vi "Process HTTP Request.vi"(8 "error in":errorcluster, 10 "id in":i32, 11 "Processing in":refnum<class "Processing.lvclass">) -> (0 "error out":errorcluster, 3 "Processing out":refnum<class "Processing.lvclass">)   [LabVIEW 2020, in "MCP Server.lvlib"]
doc: "Answers one HTTP request on the MCP endpoint following the MCP Streamable HTTP transport rules, and stores the response in the Processing object.\n\n1. ACCESS: reads the client host (Get Request, Get Client URI, Get Host: the name from a reverse DNS lookup of the client address), the local address of the connection the request arrived on (Connection Local IP.vi, no DNS) and the Authorization header, and passes them to Check Client Access.vi with the access settings Start.vi stored for this server. \"This computer only\" is decided by that local address; an error reading it only leaves it empty, which Check Client Access.vi refuses in that mode, and never turns into a 500. A client that is not allowed gets 403, a missing or wrong bearer token 401 with WWW-Authenticate: Bearer. These checks win over every later one.\n2. Reads the HTTP method and the Origin and MCP-Protocol-Version request headers and passes them to Validate HTTP Request.vi. Also reads the Mcp-Method and Mcp-Name headers (MCP 2026-07-28).\n3. Rejected request (403, 401, 405 or 400): the MCP server is NOT called. The response carries the status code and the JSON-RPC error payload with Content-Type application/json. A 405 additionally carries the header Allow: POST.\n4. Accepted request: Prepare Request Dispatch.vi answers a legacy notifications/cancelled itself and decides whether a tools/call is streamed (Start Streamed Request.vi). Otherwise the request body, one message or a batch of messages, is passed with the three MCP headers to Handle MCP Request.vi, which decides the era (legacy or modern) per request, makes the modern header checks and answers; its errors are cleared. Its status code is used: 202 with an empty body for a notification, 200 with Content-Type application/json, or 400/404 for a refused modern request.\n\nerror out reports only errors of the first two header reads. It is informational: a response is always set."
uses:
  MCP Server.lvlib
  <vilib>/IlluminatedG/IG HTTP Server/HTTP Server/Processing/Processing.lvclass
  <vilib>/IlluminatedG/IG HTTP Server/HTTP Server/Processing/Processing.lvclass/Processing.ctl
  MCP SSE Response/MCP SSE Response.lvclass
  C:/Program Files/National Instruments/LabVIEW 2026/vi.lib/IlluminatedG/IG HTTP Utils/HTTP Utils/Response/Response.lvclass
  <vilib>/IlluminatedG/IG HTTP Utils/HTTP Utils/Request/Get Method.vi
  <vilib>/IlluminatedG/IG HTTP Utils/HTTP Utils/Request/Header Value.vi
  <vilib>/IlluminatedG/IG HTTP Utils/HTTP Utils/Request/Get Body.vi
  <vilib>/IlluminatedG/IG HTTP Utils/HTTP Utils/Response/Response.lvclass
  <vilib>/IlluminatedG/lv-stream/URI/URI.lvclass
  <vilib>/IlluminatedG/IG HTTP Utils/HTTP Utils/Request/Request.lvclass
  MCP Connection Probe/MCP Connection Probe.lvclass
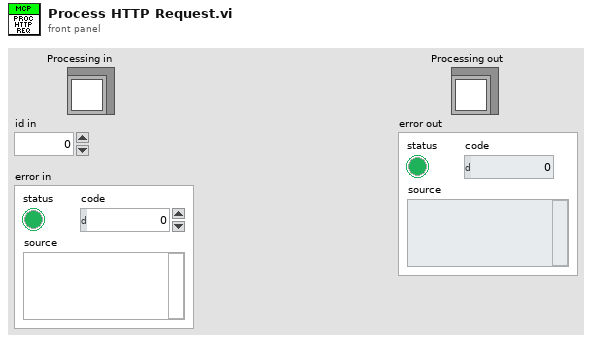
[diagram p1: front panel]
types:
  T1 = typedef "HTTP Utils.lvlib/Method.ctl" = enum16{"GET", "HEAD", "POST", "PUT", "DELETE", "CONNECT", "OPTIONS", "TRACE", "PATCH"}
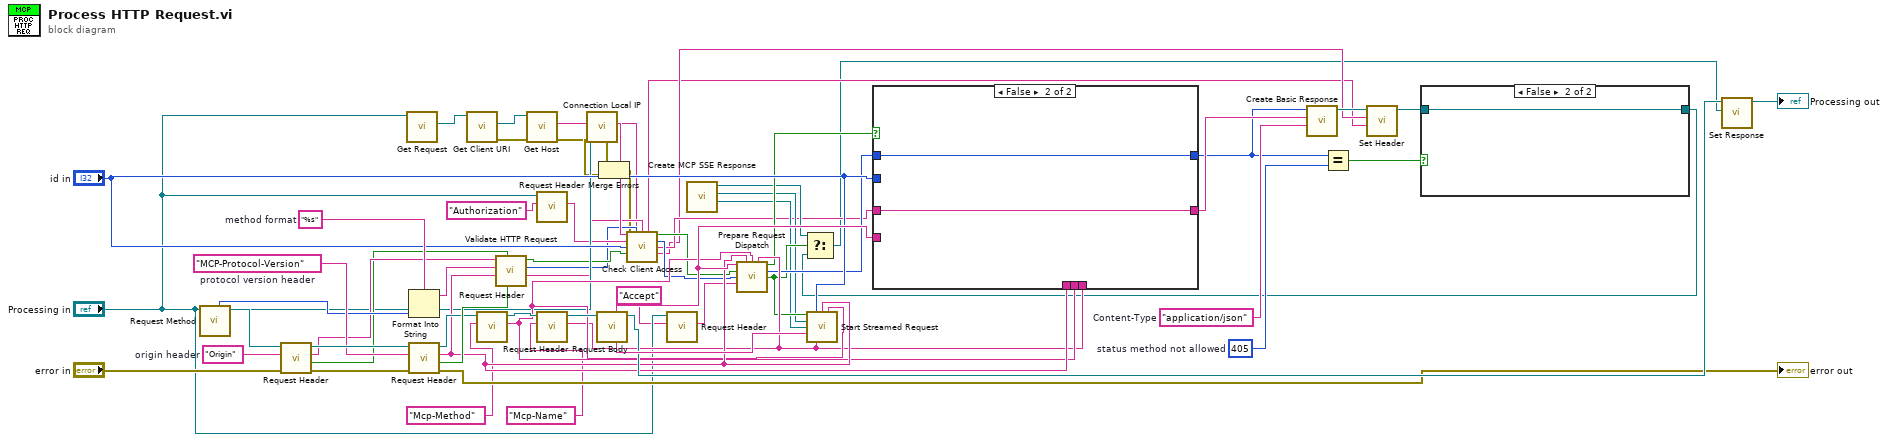
[diagram p0: block diagram]
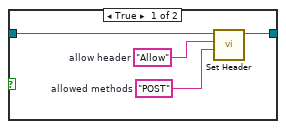
[diagram p2: hidden frame]
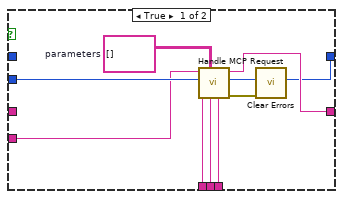
[diagram p3: hidden frame]
diagram:
  w44 = u16 405  # status method not allowed
  w46 = "application/json"  # Content-Type
  w54 = "%s"  # method format
  w57 = "MCP-Protocol-Version"  # protocol version header
  w60 = "Origin"  # origin header
  n1 = call <vilib>:"Request Method.vi"("Processing in"="Processing in") -> ("Processing out"=w61:refnum<class "Processing.lvclass">, "Request Method"=w55:T1)  [unwired: 9 in]
  n2 = call <vilib>:"Request Header.vi"("error in (no error)"="error in", "Header"=w60, "Processing in"=w61) -> ("error out"=w56:errorcluster, "Exists"=w52:bool, "Value"=w53:string, "Processing out"=w58:refnum<class "Processing.lvclass">)  [unwired: 5 in]
  n3 = call <vilib>:"Get Request.vi"("Processing in"="Processing in") -> ("Request"=w21:refnum<class "Request.lvclass">)  [unwired: 9 in, 1 out]
  n4 = Format Into String(format string=w54, w55) -> (resulting string=w51:string)  [unwired: 2 in, 1 out]
  n5 = call <vilib>:"Request Header.vi"("error in (no error)"=w56, "Header"=w57, "Processing in"=w58) -> ("error out"=→"error out":errorcluster, "Exists"=w50:bool, "Value"=w36:string, "Processing out"=w38:refnum<class "Processing.lvclass">)  [unwired: 5 in]
  n6 = call <vilib>:"Get Client URI.vi"("Request in"=w21) -> ("error out"=w19:errorcluster, "Client URI"=w20:refnum<class "URI.lvclass">)  [unwired: 8 in, 1 out]
  n7 = call <vilib>:"Request Header.vi"("Header"="Mcp-Method", "Processing in"=w38) -> ("Value"=w35:string, "Processing out"=w37:refnum<class "Processing.lvclass">)  [unwired: 6 in, 2 out]
  n8 = call "Validate HTTP Request.vi"("protocol version exists"=w50, "origin exists"=w52, "protocol version"=w36, "method"=w51, "origin"=w53) -> ("payload"=w10:string, "status code"=w11:u16, "accepted?"=w12:bool)  [unwired: 3 in, 1 out]
  n9 = call <vilib>:"Get Host.vi"("error in (no error)"=w19, "URI in"=w20) -> ("error out"=w3:errorcluster, "Host"=w18:string)  [unwired: 7 in, 1 out]
  n10 = call <vilib>:"Request Header.vi"("Header"="Authorization", "Processing in"="Processing in") -> ("Value"=w17:string)  [unwired: 6 in, 3 out]
  n11 = call <vilib>:"Request Header.vi"("Header"="Mcp-Name", "Processing in"=w37) -> ("Value"=w34:string, "Processing out"=w39:refnum<class "Processing.lvclass">)  [unwired: 6 in, 2 out]
  n12 = call "Connection Local IP.vi"("Processing in"="Processing in") -> ("error out"=w4:errorcluster, "local IP"=w1:string)  [unwired: 8 in, 1 out]
  n13 = call <vilib>:"Request Body.vi"("Processing in"=w39) -> ("Processing out"=w42:refnum<class "Processing.lvclass">, "Request Body"=w49:string)  [unwired: 9 in]
  n14 = Merge Errors(w3, w4) -> (w2:errorcluster)
  n15 = call "Check Client Access.vi"("client host"=w18, "status code"=w11, "payload"=w10, "Authorization"=w17, "id in"="id in", "accepted?"=w12, "error in"=w2, "local IP"=w1) -> ("header value"=w7:string, "accepted out"=w16:bool, "status code out"=w15:u16, "payload out"=w14:string, "header"=w8:string)  [unwired: 2 in, 1 out]
  n16 = call <vilib>:"Request Header.vi"("Header"="Accept", "Processing in"="Processing in") -> ("Value"=w30:string)  [unwired: 6 in, 3 out]
  n17 = call "Create MCP SSE Response.vi"() -> ("cancelled"=w25:refnum<queue>, "events"=w26:refnum<queue>, "MCP SSE Response out"=w22:refnum<class "MCP SSE Response.lvclass">)  [unwired: 8 in, 1 out]
  n18 = call "Prepare Request Dispatch.vi"("request"=w49, "protocol version"=w36, "Mcp-Method"=w35, "Mcp-Name"=w34, "accepted?"=w16, "status code"=w15, "Accept"=w30) -> ("accepted out"=w29:bool, "status code out"=w28:u16, "stream?"=w27:bool)  [unwired: 5 in, 1 out]
  n19 = call "Start Streamed Request.vi"("stream?"=w27, "id in"="id in", "protocol version"=w36, "Mcp-Method"=w35, "events"=w26, "cancelled"=w25, "request"=w49, "Mcp-Name"=w34) -> ()  [unwired: 7 in, 1 out]
  n20 = case shown="False" w29 {
    tunnel: w49 -> [w67 _]
    tunnel: "id in" -> [w70 _]
    tunnel: w28 -> [_ w72]
    tunnel: w14 -> [_ w71]
    tunnel: [w62 w72] -> w45
    tunnel: [w66 w71] -> w47
    tunnel: w36 -> [w65 _]
    tunnel: w35 -> [w64 _]
    tunnel: w34 -> [w63 _]
    frame True {
      w69 = string[][] []  # parameters
      n21 = call "Handle MCP Request.vi"("Mcp-Name"=w63, "Mcp-Method"=w64, "parameters"=w69, "protocol version"=w65, "id in"=w70, "request"=w67) -> ("error out"=w68:errorcluster, "status code"=w62:u16, "response"=w66:string)  [unwired: 3 in]
      n22 = call <vilib>:"Clear Errors.vi"("error in (no error)"=w68) -> ()  [unwired: 5 in, 2 out]
    }
    frame False {
    }
  }
  n23 = call <vilib>:"Create Basic Response.vi"("Content-Type (text/plain)"=w46, "Payload"=w47, "Status Code"=w45) -> ("Response out"=w9:refnum<class "Response.lvclass">)  [unwired: 7 in, 1 out]
  n24 = Equal?(x=w45, y=w44) -> (x = y?=w43:bool)
  n25 = call <vilib>:"Set Header.vi"("Value"=w7, "Header"=w8, "Response in"=w9) -> ("Response out"=w13:refnum<class "Response.lvclass">)  [unwired: 6 in, 2 out]
  n26 = case shown="False" w43 {
    tunnel: w13 -> [w76 w77]
    tunnel: [w73 w77] -> w23
    frame True {
      w74 = "POST"  # allowed methods
      w75 = "Allow"  # allow header
      n27 = call <vilib>:"Set Header.vi"("Value"=w74, "Header"=w75, "Response in"=w76) -> ("Response out"=w73:refnum<class "Response.lvclass">)  [unwired: 6 in, 2 out]
    }
    frame False {
    }
  }
  n28 = Select(t=w22, s=w27, f=w23) -> (s? t:f=w5:refnum<class "Response.lvclass">)
  n29 = call <vilib>:"Set Response.vi"("Response"=w5, "Processing in"=w42) -> ("Processing out"=→"Processing out":refnum<class "Processing.lvclass">)  [unwired: 9 in]
